vi "Autocomplete UI.vi"(0 "Allow Undefined Values? (F)":bool, 3 "Shared Options (Local)":refnum<class "Shared Options.lvclass">, 4 "LstBox Refnum":refnum<vi>, 5 "Ready Notifier":refnum<notifier>, 6 "Height (200)":i16=200, 7 "Stop Event":refnum<user-event>, 8 "Options":refnum<user-event>, 9 "Selection Event":refnum<user-event>, 10 "Autohide ListBox (F)":bool, 11 "Str Refnum":refnum<vi>) -> ()   [LabVIEW 2020, in "AutoComplete.lvlib"]
uses:
  AutoComplete.lvlib
  Shared Options/Shared Options.lvclass
  Shared Options/Shared Options.lvclass/Shared Options.ctl
  <vilib>/event_ctls.llb/eventvkey.ctl
  2bbeccc4-f5c7-4b1f-9c98-b5fc07e3c1ce.vi/ff40df25-0e41-4205-825d-56c19dc320b6.vi
  adb1b637-e644-4a2b-a889-87a49f600a6b.vi/ff40df25-0e41-4205-825d-56c19dc320b6.vi
  8bf2cb14-dd23-42fb-b25d-e931b1f6f137.vi/ff40df25-0e41-4205-825d-56c19dc320b6.vi
  38f8acc8-80ee-43c0-9cf5-b31e4ef728cb.vi/ff40df25-0e41-4205-825d-56c19dc320b6.vi
  Shared Options/Get Options.vi
  4d5de0ce-fc26-40c3-9d22-491c84d57e29.vi/ff40df25-0e41-4205-825d-56c19dc320b6.vi
  b3c8b82e-d583-48e2-9ef9-c0cafbc50cc7.vi/ff40df25-0e41-4205-825d-56c19dc320b6.vi
  7e01c71a-78f3-4c4a-84ad-b92dc33d679c.vi/ff40df25-0e41-4205-825d-56c19dc320b6.vi
  5dd5d405-7d1f-4bc1-b915-6f0a7d99e31e.vi/ff40df25-0e41-4205-825d-56c19dc320b6.vi
  be137cc3-4b0f-4398-925d-57dde7a7d9de.vi/ff40df25-0e41-4205-825d-56c19dc320b6.vi
  2350a281-22d7-49b1-b9ce-e93203cffff4.vi/ff40df25-0e41-4205-825d-56c19dc320b6.vi
  77dab034-7a2f-4536-8477-6d526260e02d.vi/ff40df25-0e41-4205-825d-56c19dc320b6.vi
  7b6c6229-26da-4fe9-8dea-dc2e91221d0d.vi/ff40df25-0e41-4205-825d-56c19dc320b6.vi
  Shared Options/Get Options.vi/8c506e71-e04c-434f-b939-6f9a1cc01d2d.vi
  Shared Options/Get Options.vi/8c506e71-e04c-434f-b939-6f9a1cc01d2d.vi/ff40df25-0e41-4205-825d-56c19dc320b6.vi
  <vilib>/Utility/Debug Log/Display.vi
panel:
  out "Revert":bool
  out "Starting Value":string
  in  "Visible":bool
  out "All Options":string[](array[string])
  in  "Listbox":i32(listbox)
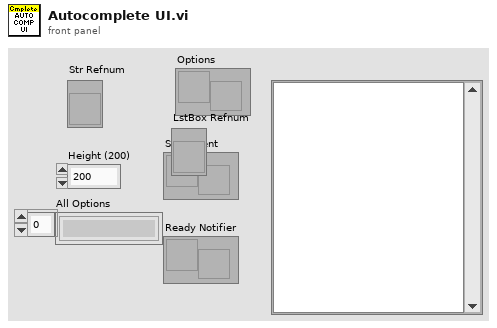
[diagram p1: front panel]
types:
  T1 = enum32{"Invalid", "Standard", "Closed", "Hidden", "Minimized", "Maximized"}
  T2 = typedef "eventvkey.ctl" = enum16{"ASCII", "Enter", "Return", "Shift", "Ctrl", "Alt", "Cmd", "Opt", "Caps", "NumLock", "Clear", "Break", "Up", "Down", "Left", "Right", "Insert", "Delete", "Home", "End", "PageUp", "PageDown", "Escape", "Help", "Pause", "ScrollLock", "F1", "F2", "F3", "F4", "F5", "F6", "F7", "F8", "F9", "F10", "F11", "F12", "F13", "F14", "F15", "F16", "F17", "F18", "F19", "F20", "F21", "F22", "F23", "F24", "Play", "VolumeUp", "VolumeDown", "Mute", "Two Byte Char"}
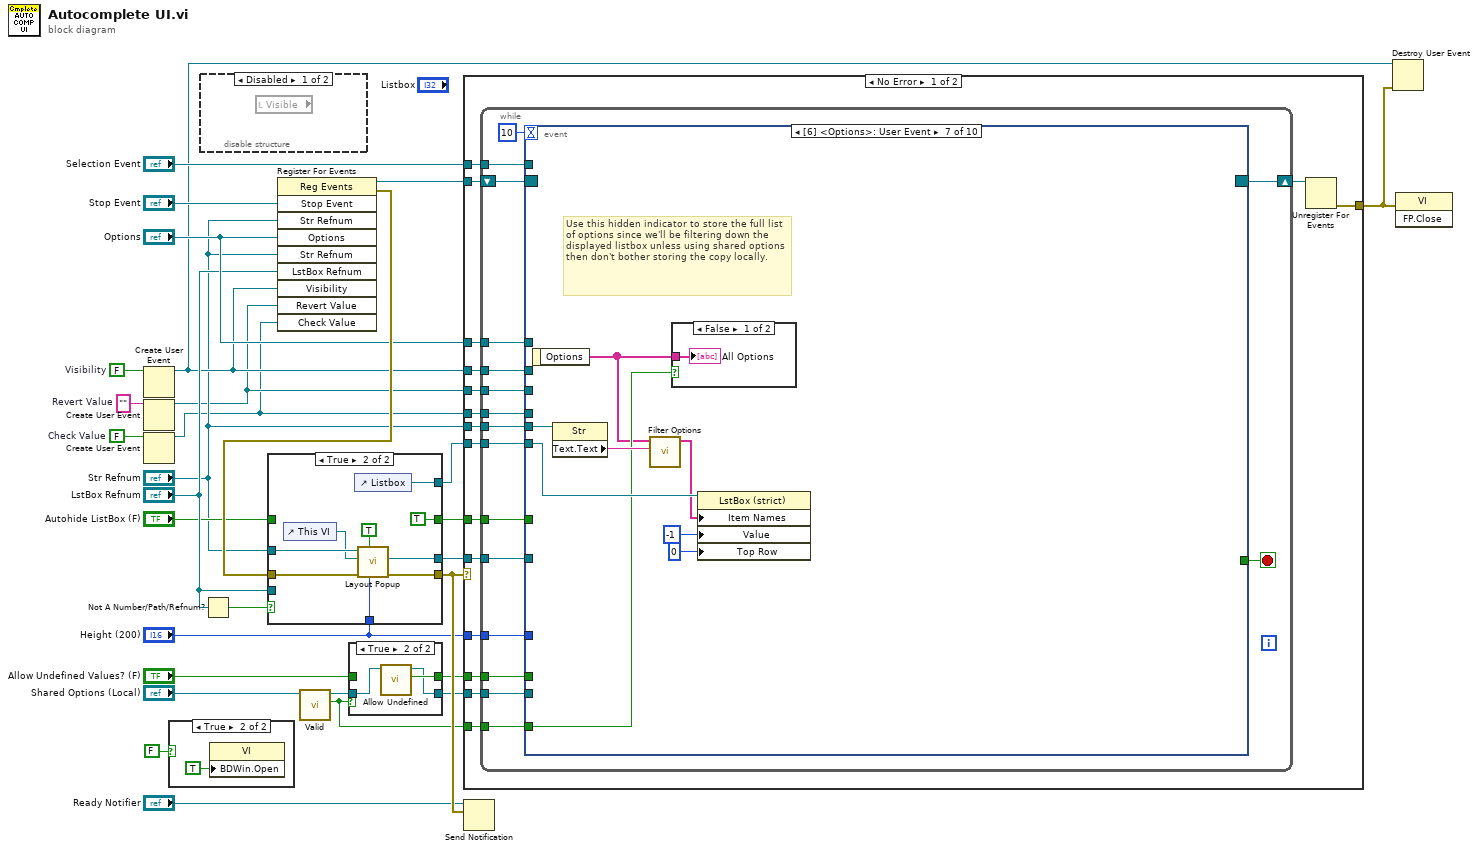
[diagram p0: block diagram]
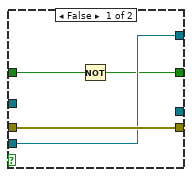
[diagram p5: hidden frame]
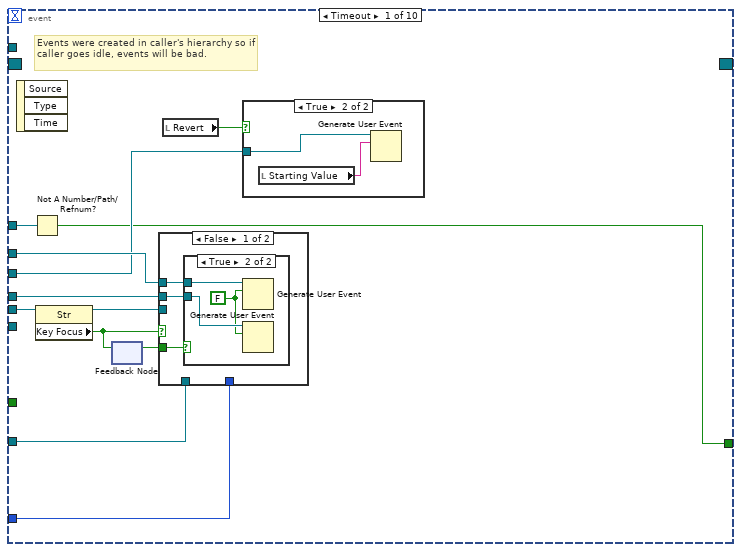
[diagram p6: hidden frame]
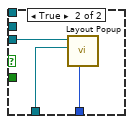
[diagram p9: hidden frame]
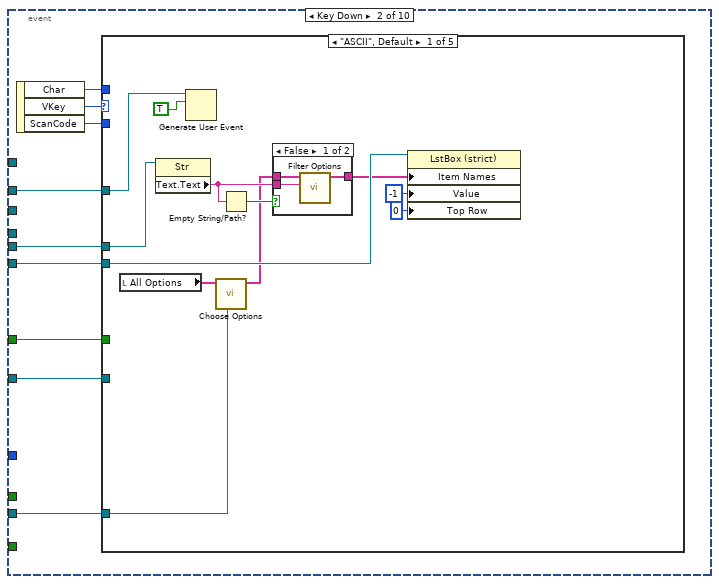
[diagram p10: hidden frame]
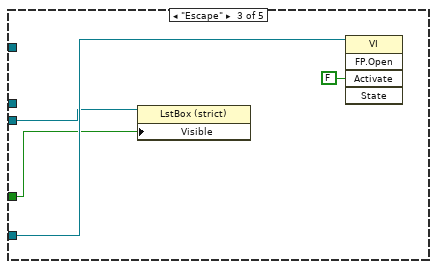
[diagram p13: hidden frame]
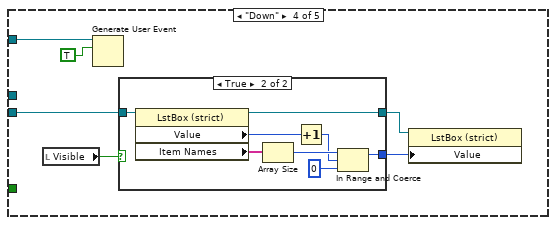
[diagram p14: hidden frame]
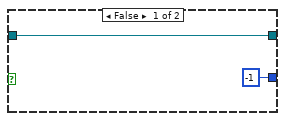
[diagram p15: hidden frame]
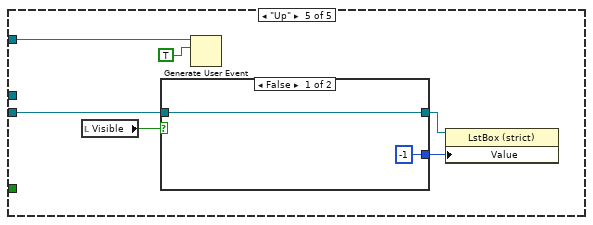
[diagram p16: hidden frame]
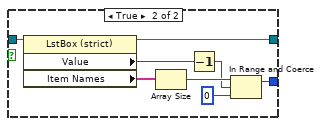
[diagram p17: hidden frame]
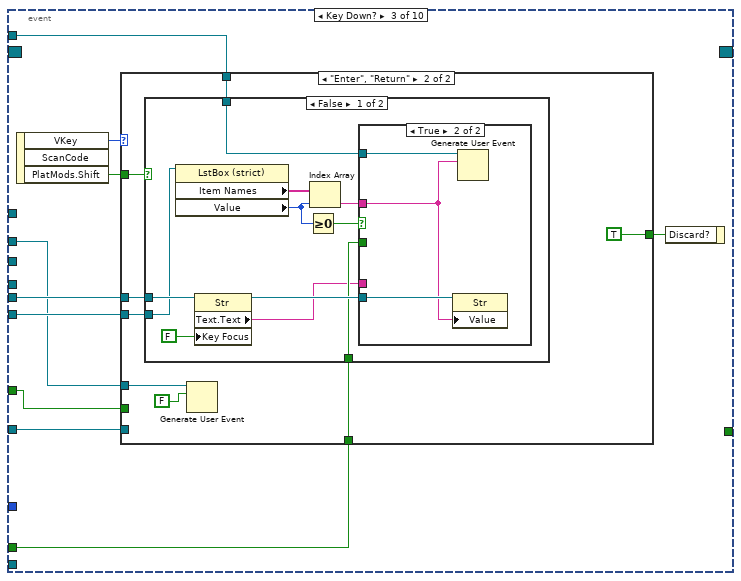
[diagram p18: hidden frame]
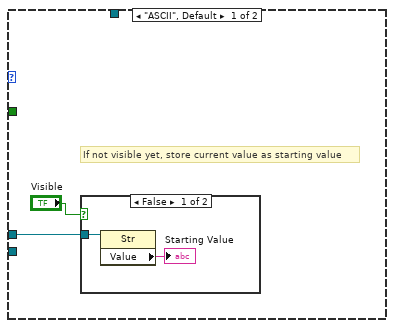
[diagram p19: hidden frame]
diagram:
  w9 = FALSE  # Check Value
  w11 = ""  # Revert Value
  w16 = FALSE  # Visibility
  n1 = Create User Event(user event datatype=w16) -> (user event=w14:refnum<user-event>)  [unwired: 1 in, 1 out]
  n2 = Create User Event(user event datatype=w11) -> (user event=w10:refnum<user-event>)  [unwired: 1 in, 1 out]
  n3 = Create User Event(user event datatype=w9) -> (user event=w8:refnum<user-event>)  [unwired: 1 in, 1 out]
  n4 = case shown="True" FALSE {
    frame False {
    }
    frame True {
      n5 = property class="VI"("BDWin.Open"=TRUE ("Block Diagram Window:Open")) -> ()  [unwired: 2 in, 2 out]
    }
  }
  n6 = disable-structure shown="Disabled" {
    frame Disabled {
      n7 = local read "Visible"() -> ()  [unwired: 1 out]
    }
    frame Enabled {
    }
  }
  n8 = Not A Number/Path/Refnum?(number/path/refnum="LstBox Refnum") -> (NaN/Path/Refnum?=w22:bool)
  n9 = register-events("Stop Event", "Str Refnum", "Options", "Str Refnum", "LstBox Refnum", w14, w10, w8) -> (reference out=w27:refnum<event-registration>, error out=w28:errorcluster)  [unwired: 2 in]
  n10 = case shown="True" w22 {
    tunnel: w28 -> [w34 w37]
    tunnel: "Height (200)" -> [_ w39]
    tunnel: [_ w36] -> w26
    tunnel: [w34 w43] -> w29
    tunnel: "Str Refnum" -> [_ w40]
    tunnel: "LstBox Refnum" -> [w33 _]
    tunnel: [w33 w42] -> w21
    tunnel: [w31 TRUE] -> w20
    tunnel: "Autohide ListBox (F)" -> [w32 _]
    frame False {
      n11 = Not(x=w32) -> (.not. x?=w31:bool)
    }
    frame True {
      n12 = control-ref of="This VI"() -> (w38:refnum<vi>)
      n13 = control-ref of="Listbox"() -> (w42:refnum<vi>)
      n14 = call "Layout Popup.vi"("Height (200)"=w39, "Initial? (F)"=TRUE, "error in (no error)"=w37, "Popup VI In"=w38, "String Control In"=w40) -> ("error out"=w43:errorcluster, "Popup VI"=w36:refnum<vi>)  [unwired: 4 in, 1 out]
    }
  }
  n15 = call "Valid.vi"("Shared Options in"="Shared Options (Local)") -> ("Valid"=w3:bool, "Shared Options out"=w5:refnum<class "Shared Options.lvclass">)  [unwired: 8 in, 1 out]
  n16 = case shown="True" w3 {
    tunnel: "Allow Undefined Values? (F)" -> [w44 _]
    tunnel: w5 -> [_ w47]
    tunnel: [_ w45] -> w4
    tunnel: [w44 w46] -> w2
    frame False {
    }
    frame True {
      n17 = call "Allow Undefined.vi"("Shared Options in"=w47) -> ("Allow Undefined Values"=w46:bool, "Shared Options out"=w45:refnum<class "Shared Options.lvclass">)  [unwired: 8 in, 1 out]
    }
  }
  n18 = case shown="No Error" w29 {
    tunnel: w27 -> [w63 _]
    tunnel: "Str Refnum" -> [w62 _]
    tunnel: [w60 _] -> w15
    tunnel: w26 -> [w59 _]
    tunnel: "Options" -> [w58 _]
    tunnel: w21 -> [w57 _]
    tunnel: w20 -> [w56 _]
    tunnel: "Selection Event" -> [w55 _]
    tunnel: w14 -> [w54 _]
    tunnel: "Height (200)" -> [w53 _]
    tunnel: w2 -> [w52 _]
    tunnel: w10 -> [w51 _]
    tunnel: w8 -> [w50 _]
    tunnel: w4 -> [w49 _]
    tunnel: w3 -> [w48 _]
    frame No Error {
      n19 = while {
        shift-right: [w79] -> w61
        shift-left: w63 -> [w80]
        tunnel: w62 -> [w77]
        tunnel: w59 -> [w75]
        tunnel: w58 -> [w74]
        tunnel: w57 -> [w73]
        tunnel: w56 -> [w72]
        tunnel: w55 -> [w71]
        tunnel: w54 -> [w70]
        tunnel: w53 -> [w69]
        tunnel: w52 -> [w68]
        tunnel: w51 -> [w67]
        tunnel: w50 -> [w66]
        tunnel: w49 -> [w65]
        tunnel: w48 -> [w64]
        stop <- w78 stop-if-true
        n20 = event shown="[6] <Options>: User Event" {
          selector: w80 -> [_ _ _ _ _ _ _ _ _ _]
          dyn-events: [_ _ _ _ _ _ _ _ _ _] -> w79
          timeout: 10 -> [_ _ _ _ _ _ _ _ _ _]
          tunnel: [w81 _ _ _ _ TRUE _ _ _ _] -> w78
          tunnel: w77 -> [w92 w112 w172 w212 w224 _ w254 w259 w270 _]
          tunnel: w75 -> [w87 w109 w171 _ w227 _ _ _ _ _]
          tunnel: w74 -> [w91 _ _ _ _ w243 _ _ _ _]
          tunnel: w73 -> [_ w108 w170 _ w226 w246 w253 _ w269 _]
          tunnel: w72 -> [_ w107 w169 _ w225 w245 _ _ _ _]
          tunnel: w71 -> [_ _ w168 w211 _ w242 _ _ w268 _]
          tunnel: w70 -> [w90 w106 w167 w209 _ w244 _ _ _ _]
          tunnel: w69 -> [w86 _ _ _ w223 _ _ _ _ _]
          tunnel: w68 -> [_ _ w166 w207 _ _ _ _ w267 _]
          tunnel: w67 -> [w85 _ _ _ _ w241 _ _ _ _]
          tunnel: w66 -> [w82 _ _ _ _ _ _ _ _ _]
          tunnel: w65 -> [_ w105 _ _ _ _ _ _ _ _]
          tunnel: w64 -> [_ _ _ _ _ w240 w250 _ _ _]
          event Timeout {
            # "Events were created in caller's hierarchy so if caller goes idle, events will be bad."
            n21 = event-data() -> ()  [unwired: 1 in, 3 out]
            n22 = Not A Number/Path/Refnum?(number/path/refnum=w91) -> (NaN/Path/Refnum?=w81:bool)
            n23 = property class="Str"(reference=w92) -> (reference out=w83:refnum<vi>, "Key Focus"=w89:bool)  [unwired: 1 in, 1 out]
            n24 = feedback-in #1(w89) -> ()
            n25 = feedback #1() -> (w88:bool)  [unwired: 1 in]
            n26 = case shown="False" w89 {
              tunnel: w90 -> [w97 _]
              tunnel: w88 -> [w96 _]
              tunnel: w83 -> [_ w103]
              tunnel: w87 -> [_ w102]
              tunnel: w86 -> [_ w101]
              tunnel: w82 -> [w95 _]
              frame False {
                n27 = case shown="True" w96 {
                  tunnel: w97 -> [_ w100]
                  tunnel: w95 -> [_ w99]
                  frame False {
                  }
                  frame True {
                    w98 = FALSE ("event data")
                    n28 = Generate User Event(user event=w100, event data cluster=w98) -> ()  [unwired: 2 in, 2 out]
                    n29 = Generate User Event(user event=w99, event data cluster=w98) -> ()  [unwired: 2 in, 2 out]
                  }
                }
              }
              frame True {
                n30 = call "Layout Popup.vi"("Height (200)"=w101, "Popup VI In"=w102, "String Control In"=w103) -> ()  [unwired: 6 in, 3 out]
              }
            }
            n31 = local read "Revert"() -> (w84:bool)
            n32 = case shown="True" w84 {
              tunnel: w85 -> [_ w94]
              frame False {
              }
              frame True {
                n33 = local read "Starting Value"() -> (w93:string)
                n34 = Generate User Event(user event=w94, event data cluster=w93) -> ()  [unwired: 2 in, 2 out]
              }
            }
          }
          event Key Down {
            n35 = event-data() -> ("Char"=w111:i16, "VKey"=w104:T2, "ScanCode"=w110:i16)  [unwired: 1 in]
            n36 = case shown="\"ASCII\", Default" w104 {
              tunnel: w112 -> [w123 _ _ _ _]
              tunnel: w111 -> [_ _ _ _ _]
              tunnel: w110 -> [_ _ _ _ _]
              tunnel: w109 -> [_ _ w131 _ _]
              tunnel: w108 -> [w118 _ w130 w137 w152]
              tunnel: w107 -> [_ _ w129 _ _]
              tunnel: w106 -> [w117 _ _ w134 w150]
              tunnel: w105 -> [w114 _ _ _ _]
              frame "ASCII", Default {
                n37 = local read "All Options"() -> (w121:string[])
                n38 = property class="Str"(reference=w123) -> ("Text.Text"=w120:string)  [unwired: 1 in, 2 out]
                n39 = Generate User Event(user event=w117, event data cluster=TRUE ("event data")) -> ()  [unwired: 2 in, 2 out]
                n40 = call "Choose Options.vi"("Shared Options"=w114, "Local Options"=w121) -> ("Options"=w115:string[])  [unwired: 9 in]
                n41 = Empty String/Path?(string/path=w120) -> (empty?=w119:bool)
                n42 = case shown="False" w119 {
                  tunnel: [w125 w128] -> w113
                  tunnel: w115 -> [w127 w128]
                  tunnel: w120 -> [w126 _]
                  frame False {
                    n43 = call "Filter Options.vi"("Text"=w126, "All Options"=w127) -> ("Filtered Names"=w125:string[])  [unwired: 9 in]
                  }
                  frame True {
                  }
                }
                n44 = property on="Property Node" class="LstBox (strict)"(reference=w118, "Item Names"=w113, "Value"=-1 ("Listbox"), "Top Row"=0) -> ()  [unwired: 1 in, 2 out]
              }
              frame "Enter", "Return" {
                # "Handled in Key Down?"
              }
              frame "Escape" {
                n45 = property class="LstBox (strict)"(reference=w130, "Visible"=w129) -> ()  [unwired: 1 in, 2 out]
                n46 = invoke class="VI" method="FP.Open"(reference=w131, "Activate"=FALSE ("Activate?")) -> ()  [unwired: 3 in, 5 out]
              }
              frame "Down" {
                n47 = local read "Visible"() -> (w133:bool)
                n48 = Generate User Event(user event=w134, event data cluster=TRUE ("event data")) -> ()  [unwired: 2 in, 2 out]
                n49 = case shown="True" w133 {
                  tunnel: [-1 ("lower limit") w143] -> w138
                  tunnel: w137 -> [w140 w142]
                  tunnel: [w140 w141] -> w136
                  frame False {
                  }
                  frame True {
                    n50 = property on="Property Node" class="LstBox (strict)"(reference=w142) -> (reference out=w141:refnum<vi>, "Value"=w147:i32, "Item Names"=w148:string[])  [unwired: 1 in, 1 out]
                    n51 = Array Size(array=w148) -> (size(s)=w146:i32)
                    n52 = Increment(x=w147) -> (x+1=w145:i32)
                    n53 = In Range and Coerce(upper limit=w146, x=w145, lower limit=0) -> (coerced(x)=w143:i32)  [unwired: 1 out]
                  }
                }
                n54 = property on="Property Node" class="LstBox (strict)"(reference=w136, "Value"=w138) -> ()  [unwired: 1 in, 2 out]
              }
              frame "Up" {
                n55 = local read "Visible"() -> (w149:bool)
                n56 = case shown="False" w149 {
                  tunnel: [-1 ("lower limit") w159] -> w154
                  tunnel: [w156 w158] -> w153
                  tunnel: w152 -> [w156 w157]
                  frame False {
                  }
                  frame True {
                    n57 = property on="Property Node" class="LstBox (strict)"(reference=w157) -> (reference out=w158:refnum<vi>, "Value"=w163:i32, "Item Names"=w164:string[])  [unwired: 1 in, 1 out]
                    n58 = Array Size(array=w164) -> (size(s)=w162:i32)
                    n59 = Decrement(x=w163) -> (x-1=w161:i32)
                    n60 = In Range and Coerce(upper limit=w162, x=w161, lower limit=0) -> (coerced(x)=w159:i32)  [unwired: 1 out]
                  }
                }
                n61 = Generate User Event(user event=w150, event data cluster=TRUE ("event data")) -> ()  [unwired: 2 in, 2 out]
                n62 = property on="Property Node" class="LstBox (strict)"(reference=w153, "Value"=w154) -> ()  [unwired: 1 in, 2 out]
              }
            }
          }
          event Key Down? {
            n63 = event-data() -> ("VKey"=w165:T2, "PlatMods.Shift"=w174:bool)  [unwired: 1 in, 1 out]
            n64 = case shown="\"Enter\", \"Return\"" w165 {
              tunnel: w174 -> [_ w186]
              tunnel: [_ TRUE] -> w173
              tunnel: w172 -> [w176 w184]
              tunnel: w171 -> [_ _]
              tunnel: w170 -> [_ w183]
              tunnel: w169 -> [_ _]
              tunnel: w168 -> [_ w182]
              tunnel: w167 -> [_ w181]
              tunnel: w166 -> [_ w179]
              frame "ASCII", Default {
                # "If not visible yet, store current value as starting value"
                n65 = case shown="False" "Visible" {
                  tunnel: w176 -> [w178 _]
                  frame False {
                    n66 = property class="Str"(reference=w178) -> ("Value"=→"Starting Value":string)  [unwired: 1 in, 2 out]
                  }
                  frame True {
                  }
                }
              }
              frame "Enter", "Return" {
                n67 = case shown="False" w186 {
                  tunnel: w184 -> [w193 _]
                  tunnel: w183 -> [w191 _]
                  tunnel: w182 -> [w190 _]
                  tunnel: w179 -> [w188 _]
                  frame False {
                    n68 = property on="Property Node" class="LstBox (strict)"(reference=w191) -> ("Item Names"=w197:string[], "Value"=w196:i32)  [unwired: 1 in, 2 out]
                    n69 = property class="Str"(reference=w193, "Key Focus"=FALSE) -> (reference out=w192:refnum<vi>, "Text.Text"=w187:string)  [unwired: 1 in, 1 out]
                    n70 = Greater Or Equal To 0?(x=w196) -> (x >= 0?=w189:bool)
                    n71 = Index Array(array=w197, index=w196) -> (element=w195:string)
                    n72 = case shown="True" w189 {
                      tunnel: w195 -> [_ w204]
                      tunnel: w192 -> [w198 w206]
                      tunnel: w190 -> [w199 w205]
                      tunnel: w188 -> [w200 _]
                      tunnel: w187 -> [w201 _]
                      frame False {
                        n73 = case shown="True" w200 {
                          tunnel: w201 -> [_ w202]
                          tunnel: w199 -> [_ w203]
                          tunnel: w198 -> [_ _]
                          frame False {
                            (unwired) TRUE ("Revert")
                          }
                          frame True {
                            n74 = Generate User Event(user event=w203, event data cluster=w202) -> ()  [unwired: 2 in, 2 out]
                          }
                        }
                      }
                      frame True {
                        n75 = property class="Str"(reference=w206, "Value"=w204) -> ()  [unwired: 1 in, 2 out]
                        n76 = Generate User Event(user event=w205, event data cluster=w204) -> ()  [unwired: 2 in, 2 out]
                      }
                    }
                  }
                  frame True {
                  }
                }
                n77 = Generate User Event(user event=w181, event data cluster=FALSE ("event data")) -> ()  [unwired: 2 in, 2 out]
              }
            }
            n78 = event-data("Discard?"=w173) -> ()  [unwired: 1 in, 1 out]
          }
          event "Listbox": Value Change {
            n79 = event-data() -> ("CtlRef"=w210:refnum<vi>)  [unwired: 1 in]
            n80 = property on="Property Node" class="LstBox (strict)"(reference=w210) -> ("Item Names"=w216:string[], "Value"=w215:i32)  [unwired: 1 in, 2 out]
            n81 = Greater Or Equal To 0?(x=w215) -> (x >= 0?=w214:bool)
            n82 = Index Array(array=w216, index=w215) -> (element=w213:string)
            n83 = Or(x=w214, y=w207) -> (x .or. y?=w208:bool)
            n84 = case shown="True" w208 {
              tunnel: w213 -> [_ w221]
              tunnel: w212 -> [_ w220]
              tunnel: w211 -> [_ w219]
              tunnel: w209 -> [_ w218]
              frame False {
              }
              frame True {
                n85 = property class="Str"(reference=w220, "Value"=w221) -> ()  [unwired: 1 in, 2 out]
                n86 = Generate User Event(user event=w219, event data cluster=w221) -> ()  [unwired: 2 in, 2 out]
                n87 = Generate User Event(user event=w218, event data cluster=FALSE ("event data")) -> ()  [unwired: 2 in, 2 out]
              }
            }
          }
          event User Event {
            n88 = event-data() -> ("Visibility"=w222:bool)  [unwired: 1 in, 4 out]
            n89 = case shown="True" w222 {
              tunnel: w227 -> [w229 w234]
              tunnel: w226 -> [w231 w238]
              tunnel: w225 -> [w228 _]
              tunnel: w224 -> [_ w235]
              tunnel: w223 -> [_ w236]
              frame False {
                (unwired) FALSE
                n90 = property class="LstBox (strict)"(reference=w231, "Visible"=w228) -> ()  [unwired: 1 in, 2 out]
                n91 = invoke class="VI" method="FP.Open"(reference=w229, "Activate"=FALSE ("Activate?"), "State"=T1."Hidden") -> ()  [unwired: 2 in, 5 out]
              }
              frame True {
                n92 = property class="LstBox (strict)"(reference=w238, "Visible"=TRUE) -> ()  [unwired: 1 in, 2 out]
                n93 = call "Layout Popup.vi"("Height (200)"=w236, "Popup VI In"=w234, "String Control In"=w235) -> ()  [unwired: 6 in, 3 out]
                n94 = invoke class="VI" method="FP.Open"(reference=w234, "Activate"=FALSE ("Activate?"), "State"=T1."Standard") -> ()  [unwired: 2 in, 5 out]
              }
            }
            n95 = local write "Visible"(w222) -> ()
          }
          event User Event {
            n96 = event-data() -> ()  [unwired: 1 in, 1 out]
            n97 = Destroy User Event(user event=w242) -> ()  [unwired: 1 in, 1 out]
            n98 = Destroy User Event(user event=w241) -> ()  [unwired: 1 in, 1 out]
            n99 = Destroy User Event(user event=w244) -> ()  [unwired: 1 in, 1 out]
            n100 = case shown="False" w240 {
              tunnel: w243 -> [w248 _]
              frame False {
                n101 = Destroy User Event(user event=w248) -> ()  [unwired: 1 in, 1 out]
              }
              frame True {
                # "Don't close options event if using shared options."
              }
            }
            n102 = property class="LstBox (strict)"(reference=w246, "Visible"=w245) -> ()  [unwired: 1 in, 2 out]
          }
          event User Event {
            # "Use this hidden indicator to store the full list of options since we'll be filtering down the displayed listbox unless using shared options then don't bother storing the copy locally."
            n103 = event-data() -> ("Options"=w249:string[])  [unwired: 1 in]
            n104 = property class="Str"(reference=w254) -> ("Text.Text"=w252:string)  [unwired: 1 in, 2 out]
            n105 = call "Filter Options.vi"("Text"=w252, "All Options"=w249) -> ("Filtered Names"=w251:string[])  [unwired: 9 in]
            n106 = case shown="False" w250 {
              tunnel: w249 -> [w257 _]
              frame False {
                "All Options" <- w257
              }
              frame True {
              }
            }
            n107 = property on="Property Node" class="LstBox (strict)"(reference=w253, "Item Names"=w251, "Value"=-1 ("Listbox"), "Top Row"=0) -> ()  [unwired: 1 in, 2 out]
          }
          event User Event {
            n108 = event-data() -> ("Revert Value"=w258:string)  [unwired: 1 in]
            n109 = property class="Str"(reference=w259, "Value"=w258) -> ()  [unwired: 1 in, 2 out]
            n110 = call <vilib>:"Beep.vi"() -> ()  [unwired: 12 in]
          }
          event User Event {
            n111 = event-data() -> ()  [unwired: 1 in, 1 out]
            n112 = property on="Property Node" class="LstBox (strict)"(reference=w269) -> ("Item Names"=w260:string[], "Value"=w266:i32)  [unwired: 1 in, 2 out]
            n113 = property class="Str"(reference=w270, "Key Focus"=FALSE) -> (reference out=w263:refnum<vi>, "Text.Text"=w261:string)  [unwired: 1 in, 1 out]
            n114 = Index Array(array=w260, index=w266) -> (element=w265:string)
            n115 = Greater Or Equal To 0?(x=w266) -> (x >= 0?=w262:bool)
            n116 = case shown="False" w262 {
              tunnel: w265 -> [_ w286]
              tunnel: w263 -> [w272 w288]
              tunnel: w268 -> [w273 w287]
              tunnel: w267 -> [w274 _]
              tunnel: w261 -> [w275 _]
              tunnel: w260 -> [w271 _]
              frame False {
                n117 = case shown="False" w274 {
                  tunnel: w275 -> [w276 w284]
                  tunnel: w273 -> [w277 w285]
                  tunnel: w272 -> [_ _]
                  tunnel: w271 -> [w280 _]
                  frame False {
                    n118 = Search 1D Array(1D array=w280, element=w276) -> (index of element=w279:i32)  [unwired: 1 in]
                    n119 = Less Than 0?(x=w279) -> (x < 0?=w278:bool)
                    n120 = case shown="True" w278 {
                      tunnel: w277 -> [w282 _]
                      tunnel: w276 -> [w281 _]
                      frame False {
                        n121 = Generate User Event(user event=w282, event data cluster=w281) -> ()  [unwired: 2 in, 2 out]
                      }
                      frame True {
                        "Revert" <- TRUE ("Revert")
                      }
                    }
                  }
                  frame True {
                    n122 = Generate User Event(user event=w285, event data cluster=w284) -> ()  [unwired: 2 in, 2 out]
                  }
                }
              }
              frame True {
                n123 = property class="Str"(reference=w288, "Value"=w286) -> ()  [unwired: 1 in, 2 out]
                n124 = Generate User Event(user event=w287, event data cluster=w286) -> ()  [unwired: 2 in, 2 out]
              }
            }
          }
          event Key Down {
            n125 = event-data() -> ("VKey"=w290:T2)  [unwired: 1 in]
            n126 = Equal?(x=w290, y=eventvkey."Escape") -> ()  [unwired: 1 out]
          }
        }
      }
      n127 = Unregister For Events(event registration refnum=w61) -> (error out=w60:errorcluster)  [unwired: 1 in]
    }
    frame Error {
    }
  }
  n128 = Send Notification(notification=w29, notifier="Ready Notifier") -> ()  [unwired: 1 in, 2 out]
  n129 = Destroy User Event(user event=w14, error in=w15) -> ()  [unwired: 1 out]
  n130 = invoke class="VI" method="FP.Close"(error in=w15) -> ()  [unwired: 2 in, 3 out]
